vi "Get Statistics.vi"(8 "error in (no error)":errorcluster, 11 "Result Model in":refnum<class "Result Model.lvclass">) -> (0 "error out":errorcluster, 2 "Results":T1)   [LabVIEW 2020, in "Result Model.lvclass"]
uses:
  Result Model/Result Model.lvclass
  Result Model/Result Model.lvclass/Result Model.ctl
  Result Model/Statistics.ctl
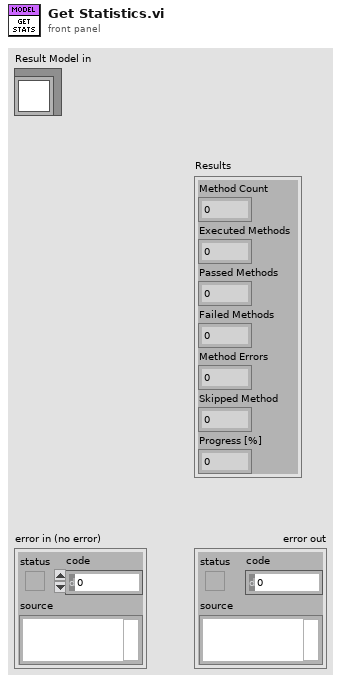
[diagram p1: front panel]
types:
  T1 = typedef "Result Model.lvclass/Statistics.ctl" = cluster{"Method Count":u32, "Executed Methods":u32, "Passed Methods":u32, "Failed Methods":u32, "Method Errors":u32, "Skipped Method":u32, "Progress [%]":dbl}
  T2 = typedef "Result.lvlib/Status.ctl" = enum16{"", "Passed", "Failed", "Error", "Skipped", "Setup Error", "Broken", "Teardown Error"}
  T3 = typedef "Result.lvlib/Type.ctl" = enum16{"Test Case", "Test Suite", "Test Run", "Pass", "Fail", "Skip", "Pass if", "Fail if", "Pass if Error", "Fail if Error", "Pass if Equal", "Fail if Equal"}
  T4 = cluster{"Tests":string[], "Run Queue":string[], "Test Statuses":map{string, T2}, "Execution Time":map{string, dbl}, "Assertions":map{string, cluster{"Result Type":T3, "Status":T2, "Description":string, "Data":cluster{"Expected":variant, "Actual":variant, "Delta":variant}}[]}}
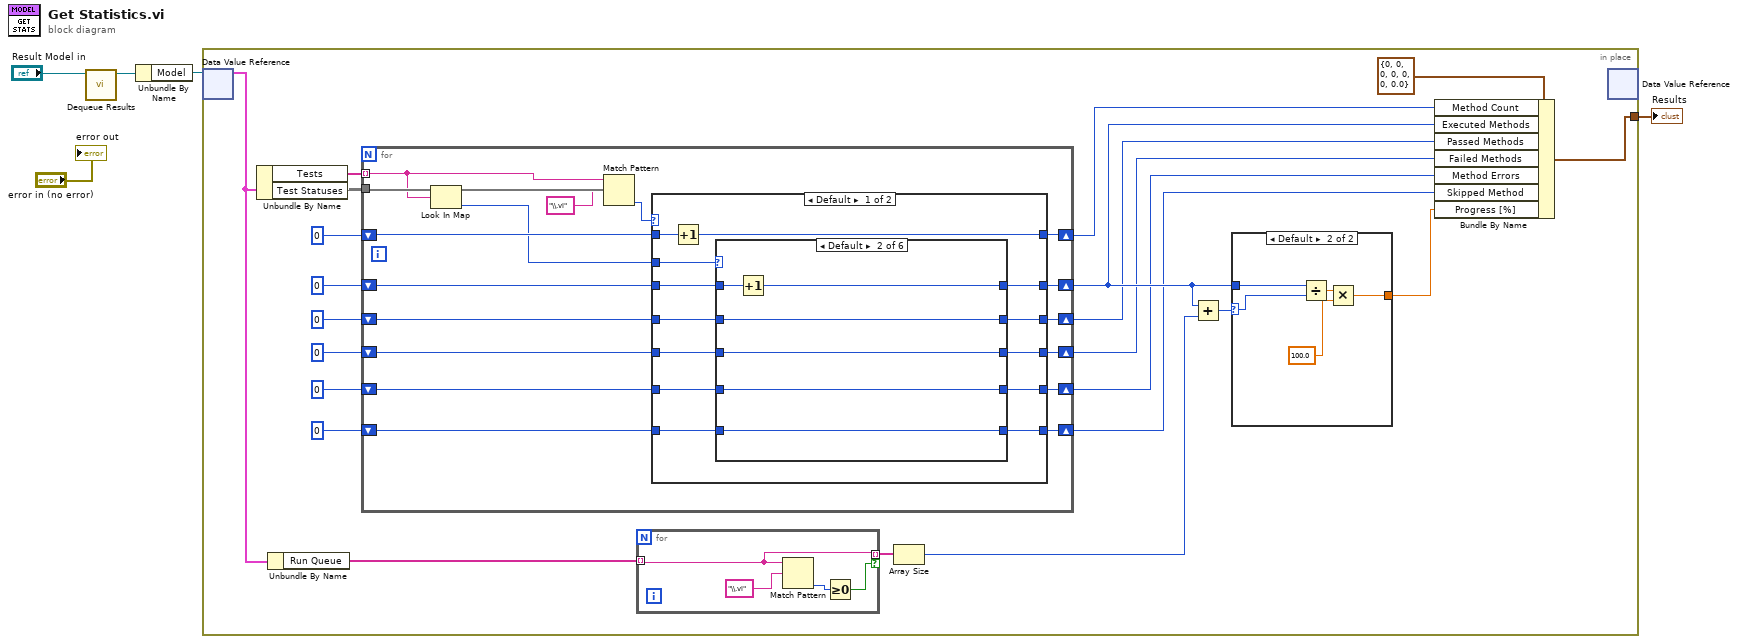
[diagram p0: block diagram]
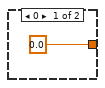
[diagram p2: hidden frame]
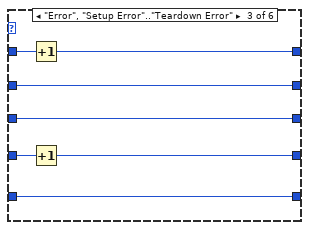
[diagram p4: hidden frame]
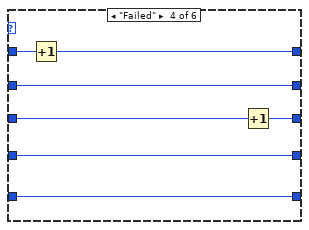
[diagram p5: hidden frame]
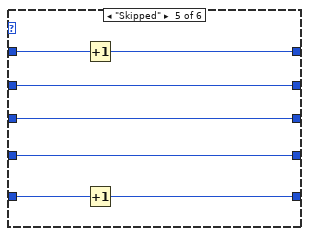
[diagram p6: hidden frame]
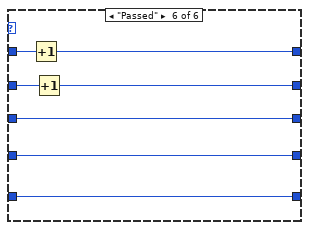
[diagram p7: hidden frame]
diagram:
  n1 = call "Dequeue Results.vi"("Result Model by Reference in"="Result Model in") -> ("Result Model by Reference out"=w2:refnum<class "Result Model.lvclass">)  [unwired: 10 in]
  n2 = Unbundle By Name(w2) -> ("Model"=w5:refnum<data-value>)
  n3 = in-place {
    in-place-border: [w26] -> w3
    n4 = in-place-dvr #1(w5) -> (w27:T4)  [unwired: 1 out]
    n5 = Unbundle By Name(w27) -> ("Tests"=w25:string[], "Test Statuses"=w23:map{string, T2})
    n6 = Unbundle By Name(w27) -> ("Run Queue"=w24:string[])
    n7 = for {
      tunnel: w23 -> [w40]
      shift-right: [w51] -> w17
      shift-left: u32 0 ("Method Count") -> [w52]
      shift-right: [w49] -> w19
      shift-left: u32 0 ("Method Count") -> [w50]
      shift-right: [w47] -> w10
      shift-left: u32 0 ("Method Count") -> [w48]
      shift-right: [w45] -> w12
      shift-left: u32 0 ("Method Count") -> [w46]
      shift-right: [w43] -> w14
      shift-left: u32 0 ("Method Count") -> [w44]
      shift-right: [w41] -> w16
      shift-left: u32 0 ("Method Count") -> [w42]
      tunnel: w25 -> [w38] mode=indexing
      n8 = Look In Map(map=w40, key=w38) -> (value=w39:T2)  [unwired: 1 in, 1 out]
      n9 = Match Pattern(string=w38, regular expression="\\.vi") -> (offset past match=w53:i32)  [unwired: 1 in, 3 out]
      n10 = case shown="Default" w53 {
        tunnel: w52 -> [w67 w112]
        tunnel: [w66 w112] -> w51
        tunnel: w39 -> [w65 _]
        tunnel: w50 -> [w64 w111]
        tunnel: [w63 w111] -> w49
        tunnel: w48 -> [w62 w110]
        tunnel: [w61 w110] -> w47
        tunnel: w46 -> [w60 w109]
        tunnel: [w59 w109] -> w45
        tunnel: w44 -> [w58 w108]
        tunnel: [w57 w108] -> w43
        tunnel: w42 -> [w56 w107]
        tunnel: [w55 w107] -> w41
        frame Default {
          n11 = Increment(x=w67) -> (x+1=w66:u32)
          n12 = case shown="Default" w65 {
            tunnel: w64 -> [w72 w78 w85 w92 w99 w106]
            tunnel: [w72 w77 w84 w91 w98 w105] -> w63
            tunnel: w62 -> [w71 w76 w83 w90 w97 w104]
            tunnel: [w71 w76 w83 w90 w97 w103] -> w61
            tunnel: w60 -> [w70 w75 w82 w89 w96 w102]
            tunnel: [w70 w75 w82 w88 w96 w102] -> w59
            tunnel: w58 -> [w69 w74 w81 w87 w95 w101]
            tunnel: [w69 w74 w80 w87 w95 w101] -> w57
            tunnel: w56 -> [w68 w73 w79 w86 w94 w100]
            tunnel: [w68 w73 w79 w86 w93 w100] -> w55
            frame "" {
            }
            frame Default {
              n13 = Increment(x=w78) -> (x+1=w77:u32)
            }
            frame "Error", "Setup Error".."Teardown Error" {
              n14 = Increment(x=w85) -> (x+1=w84:u32)
              n15 = Increment(x=w81) -> (x+1=w80:u32)
            }
            frame "Failed" {
              n16 = Increment(x=w92) -> (x+1=w91:u32)
              n17 = Increment(x=w89) -> (x+1=w88:u32)
            }
            frame "Skipped" {
              n18 = Increment(x=w99) -> (x+1=w98:u32)
              n19 = Increment(x=w94) -> (x+1=w93:u32)
            }
            frame "Passed" {
              n20 = Increment(x=w106) -> (x+1=w105:u32)
              n21 = Increment(x=w104) -> (x+1=w103:u32)
            }
          }
        }
        frame -1 {
        }
      }
    }
    n22 = for {
      tunnel: w24 -> [w29] mode=indexing
      tunnel: [w29] -> w21 mode=indexing if=w28
      n23 = Match Pattern(string=w29, regular expression="\\.vi") -> (offset past match=w30:i32)  [unwired: 1 in, 3 out]
      n24 = Greater Or Equal To 0?(x=w30) -> (x >= 0?=w28:bool)
    }
    n25 = Array Size(array=w21) -> (size(s)=w22:i32)
    n26 = Add(x=w19, y=w22) -> (x+y=w20:u32)
    n27 = case shown="Default" w20 {
      selector: w20 -> [_ w33]
      tunnel: w19 -> [_ w34]
      tunnel: [0.0 w35] -> w18
      frame 0 {
      }
      frame Default {
        n28 = Divide(x=w34, y=w33) -> (x/y=w37:dbl)
        n29 = Multiply(x=w37, y=100.0) -> (x*y=w35:dbl)
      }
    }
    n30 = Bundle By Name(cluster=T1 {"Method Count"=0, "Executed Methods"=0, "Passed Methods"=0, "Failed Methods"=0, "Method Errors"=0, "Skipped Method"=0, "Progress [%]"=0.0} ("Results"), "Method Count"=w17, "Executed Methods"=w19, "Passed Methods"=w10, "Failed Methods"=w12, "Method Errors"=w14, "Skipped Method"=w16, "Progress [%]"=w18) -> (w26:T1)
    n31 = in-place-dvr #1() -> ()  [unwired: 1 in, 2 out]
  }
  "Results" <- w3
  "error out" <- "error in (no error)"
